vi "I2C Grove 64x128OLED_SSD1315_SpinningCTI.vi"() -> ()   [LabVIEW 2020, in "CTI-Scratchpad.lvlib"]
uses:
  CTI-Scratchpad.lvlib
  CTI/Identity.ctl
  CTI/Error Reporting.ctl
  CTI/GPIO Number.ctl
  CTI/I2C Number.ctl
  dd06e040-5a0f-4774-bb4c-0085522d4b26.vi
  CTI/Session/Session.lvclass
  CTI-Peripheral/I2C OLED/64x128 I2C OLED SSD1315/64x128 I2C OLED SSD1315.lvclass
  CTI/VisaComms/VisaComms.lvclass
  CTI/CTI.lvlib
panel:
  in  "milliseconds to wait":u32=50
  out "Identity":T1
  in  "stop":bool
  out "2D Picture":picture
  in  "Grove Connector":enum16{"I2C0", "I2C1"}(ring)
  out "error out":errorcluster
  in  "Port":refnum<visa-resource-name>="COM4"
  # "Thanks to Emmanuel Geveaux!"
  # "https://wiki.seeedstudio.com/Grove-OLED-Display-0.96-SSD1315/"
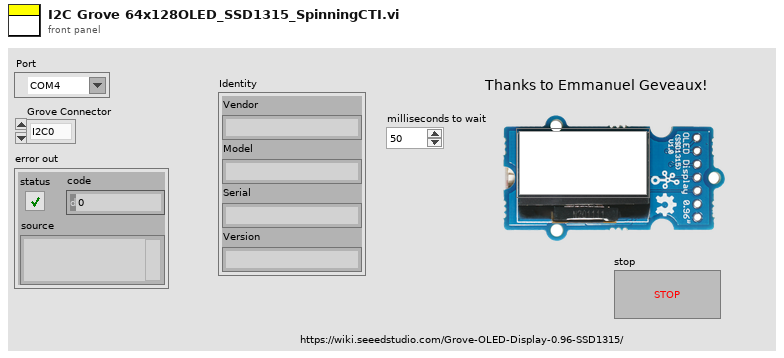
[diagram p1: front panel]
types:
  T1 = typedef "CTI.lvlib/Identity.ctl" = cluster{"Vendor":string, "Model":string, "Serial":string, "Version":string}
  T2 = typedef "CTI.lvlib/Error Reporting.ctl" = enum16{"Minimal", "Moderate", "Full"}
  T3 = typedef "CTI.lvlib/I2C Number.ctl" = i8
  T4 = typedef "CTI.lvlib/GPIO Number.ctl" = i8
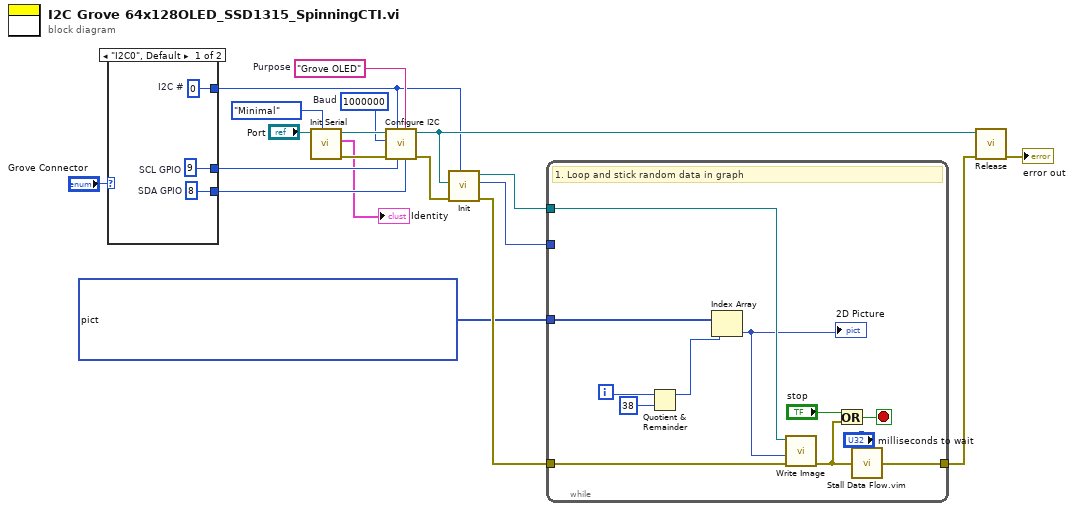
[diagram p0: block diagram]
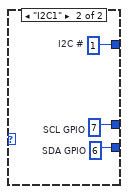
[diagram p2: hidden frame]
diagram:
  w14 = "Grove OLED"  # Purpose
  w15 = u32 1000000  # Baud
  n1 = case shown="\"I2C0\", Default" "Grove Connector" {
    tunnel: [w22 w25] -> w10
    tunnel: [w21 w24] -> w9
    tunnel: [w20 w23] -> w8
    frame "I2C0", Default {
      w20 = T3 0  # I2C #
      w21 = T4 8  # SDA GPIO
      w22 = T4 9  # SCL GPIO
    }
    frame "I2C1" {
      w23 = T3 1  # I2C #
      w24 = T4 6  # SDA GPIO
      w25 = T4 7  # SCL GPIO
    }
  }
  n2 = call "Init Serial.vi"("Error Checking (Full)"=Error_Reporting."Minimal", "VISA resource name in"="Port") -> ("error out"=w16:errorcluster, "Identity"=→"Identity":T1, "Session"=w17:refnum<class "Session.lvclass">)  [unwired: 7 in]
  n3 = call "Configure I2C.vi"("SDA GPIO"=w9, "Purpose (\"I2C\")"=w14, "SCL GPIO"=w10, "I2C #"=w8, "error in (no error)"=w16, "Baud"=w15, "Session in"=w17) -> ("error out"=w13:errorcluster, "Session out"=w12:refnum<class "Session.lvclass">)  [unwired: 3 in]
  n4 = call "Init.vi"("I2C #"=w8, "error in (no error)"=w13, "Session In"=w12) -> ("error out"=w4:errorcluster, "2D Picture"=w6:picture, "64x128 I2C OLED SSD1315 Out"=w5:refnum<class "64x128 I2C OLED SSD1315.lvclass">)  [unwired: 6 in]
  n5 = while {
    tunnel: w6 -> [_]
    tunnel: w4 -> [w36]
    tunnel: w5 -> [w37]
    tunnel: [w28] -> w3
    tunnel: picture[] [bytes[1072], bytes[1072], bytes[1072], bytes[1072], bytes[1072], bytes[1072], bytes[1072], bytes[1072], bytes[1072], bytes[1072], bytes[1072], bytes[1072], bytes[1072], bytes[1072], bytes[1072], bytes[1072], bytes[1072], bytes[1072], bytes[1072], bytes[1072], bytes[1072], bytes[1072], bytes[1072], bytes[1072], bytes[1072], bytes[1072], bytes[1072], bytes[1072], bytes[1072], bytes[1072], bytes[1072], bytes[1072], bytes[1072], bytes[1072], bytes[1072], bytes[1072], bytes[1072], bytes[1072]] ("appended array 2") -> [w29]
    i -> [w32]
    stop <- w34 stop-if-true
    # "1. Loop and stick random data in graph"
    n6 = Quotient & Remainder(x=w32, y=38) -> (x-y*floor(x/y)=w30:i32)  [unwired: 1 out]
    n7 = Index Array(array=w29, index=w30) -> (element=w26:picture)
    "2D Picture" <- w26
    n8 = call-dynamic "Write Image.vi"("error in (no error)"=w36, "2D Picture"=w26, "64x128 I2C OLED SSD1315 In"=w37) -> ("error out"=w33:errorcluster)  [unwired: 7 in, 1 out]
    n9 = Or(x="stop", y=w33) -> (x .or. y?=w34:bool)
    n10 = call "Stall Data Flow.vim"("value in"=w33, "milliseconds to wait"="milliseconds to wait") -> ("value out"=w28:errorcluster)  [unwired: 1 out]
  }
  n11 = call-dynamic "Release.vi"("error in (no error)"=w3, "Session in"=w12) -> ("error out"=→"error out":errorcluster)  [unwired: 9 in]
